vi "measure BT Hop Number.vi"(8 "error in (no error)":errorcluster, 11 "SA Measurement in":refnum<class "SA Measurement.lvclass">) -> (0 "error out":errorcluster, 3 "SA Measurement out":refnum<class "SA Measurement.lvclass">)   [LabVIEW 2023, in "Spectrum Analyzer.lvlib" / "SA Measurement.lvclass"]
uses:
  SA Measurement.lvclass
  SA Measurement.lvclass/SA Measurement.ctl
  TYPE DEFINITION/Keysight 9020A/TYPE Measurement Preset.ctl
  Spectrum Analyzer.lvlib
  TYPE DEFINITION/TYPE RBW and VBW Select.ctl
  Interface_Spectrum/Interface_Spectrum.lvclass
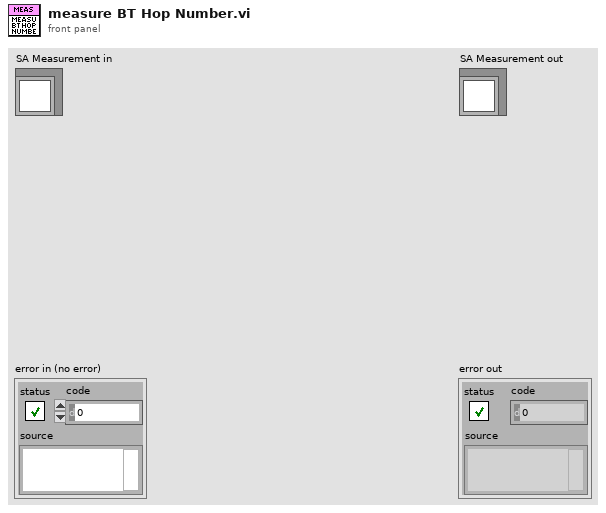
[diagram p1: front panel]
types:
  T1 = typedef "Spectrum Analyzer.lvlib/TYPE RBW and VBW Select.ctl" = enum16{"Res BW", "Video BW"}
  T2 = typedef "Spectrum Analyzer.lvlib/TYPE Measurement Preset.ctl" = enum16{"Sweep SA Mode", "Channel Power", "Occupied BW", "ACP", "Spurious Emission", "Spurious Emission Mask", "Burst Power (Transmit Power)"}
  T3 = typedef "Spectrum Analyzer.lvlib/TYPE Reference Level and Atten Param.ctl" = cluster{"Reference Level":dbl, "Atten":i32, "Atten Auto?":bool, "Reference Level Offset":dbl}
  T4 = typedef "Spectrum Analyzer.lvlib/TYPE Start and Stop Frequency.ctl" = cluster{"Start":dbl, "Stop":dbl}
  T5 = typedef "Spectrum Analyzer.lvlib/TYPE Display Trace Mode Select.ctl" = enum16{"Clear Write", "Max Hold", "Min Hold", "Average", "View"}
  T6 = typedef "Spectrum Analyzer.lvlib/TYPE Detect Mode Select.ctl" = enum16{"Det Auto (Normal)", "Auto Peak", "Positive Peak", "Negative Peak", "Sample", "RMS", "Average", "Quasipeak", "CISPR Average", "RMS Average"}
  T7 = cluster{"Trace Mode":T5, "Detector Type":T6, "Detect Auto?":bool}[]
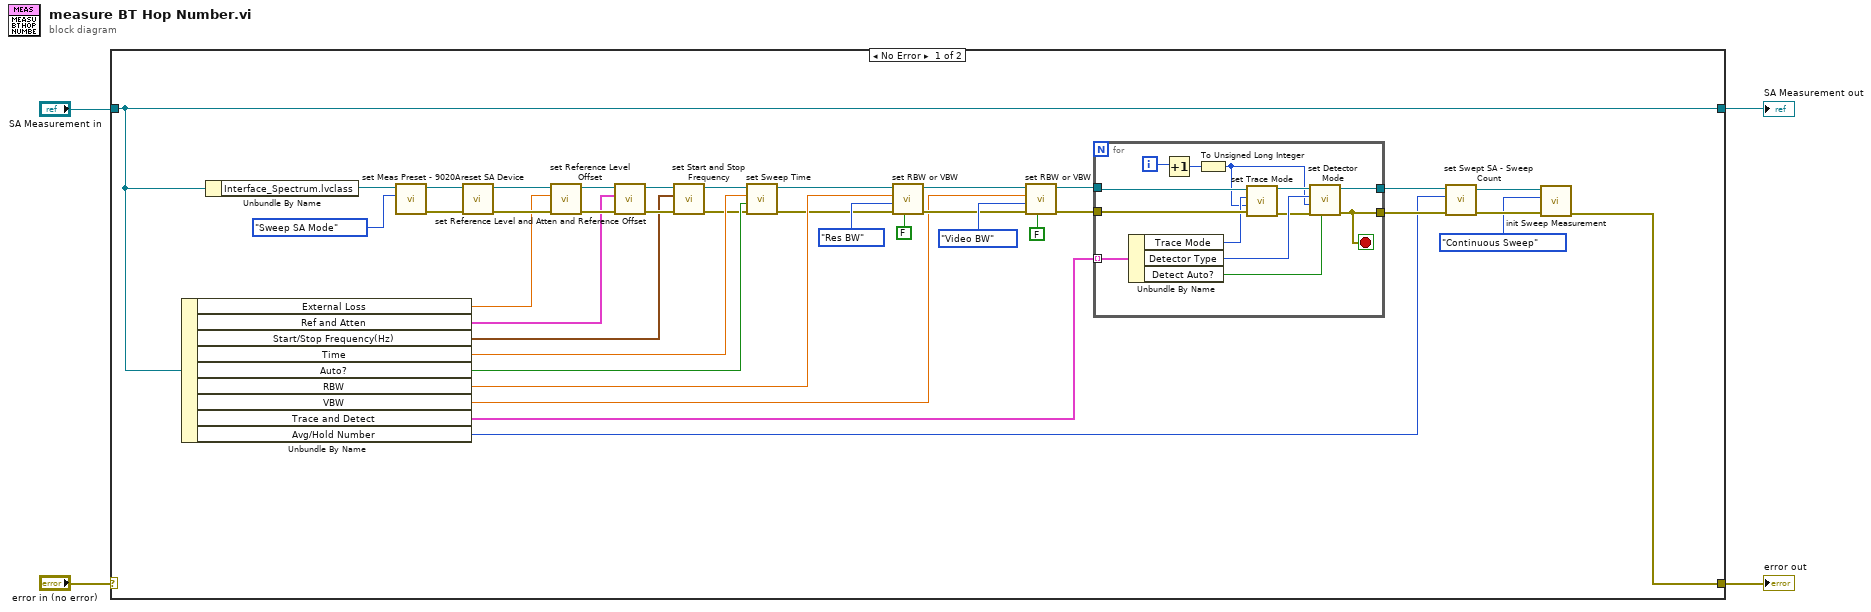
[diagram p0: block diagram]
diagram:
  n1 = case shown="No Error" "error in (no error)" {
    selector: "error in (no error)" -> [_ w57]
    tunnel: [w5 w57] -> w1
    tunnel: [w6 w56] -> w2
    tunnel: "SA Measurement in" -> [w6 w56]
    frame No Error {
      n2 = Unbundle By Name(w6) -> ("External Loss"=w34:dbl, "Ref and Atten"=w33:T3, "Start/Stop Frequency(Hz)"=w12:T4, "Time"=w18:dbl, "Auto?"=w17:bool, "RBW"=w26:dbl, "VBW"=w25:dbl, "Trace and Detect"=w22:T7, "Avg/Hold Number"=w19:u32)
      n3 = Unbundle By Name(w6) -> ("Interface_Spectrum.lvclass"=w42:refnum<class "Interface_Spectrum.lvclass">)
      n4 = call-dynamic "set Meas Preset - 9020A.vi"("Measurement Preset"=TYPE_Measurement_Preset."Sweep SA Mode", "Interface_Spectrum in"=w42) -> ("error out"=w39:errorcluster, "Interface_Spectrum out"=w40:refnum<class "Interface_Spectrum.lvclass">)  [unwired: 8 in]
      n5 = call-dynamic "reset SA Device.vi"("error in (no error)"=w39, "Interface_Spectrum in"=w40) -> ("error out"=w37:errorcluster, "Interface_Spectrum out"=w38:refnum<class "Interface_Spectrum.lvclass">)  [unwired: 8 in]
      n6 = call-dynamic "set Reference Level Offset.vi"("error in (no error)"=w37, "Reference Level Offset"=w34, "Interface_Spectrum in"=w38) -> ("error out"=w35:errorcluster, "Interface_Spectrum out"=w36:refnum<class "Interface_Spectrum.lvclass">)  [unwired: 7 in]
      n7 = call-dynamic "set Reference Level and Atten and Reference Offset.vi"("error in (no error)"=w35, "Reference Level, Atten, Reference Offset"=w33, "Interface_Spectrum in"=w36) -> ("error out"=w13:errorcluster, "Interface_Spectrum out"=w14:refnum<class "Interface_Spectrum.lvclass">)  [unwired: 7 in]
      n8 = call-dynamic "set Start and Stop Frequency.vi"("error in (no error)"=w13, "Start/Stop Frequency(Hz)"=w12, "Interface_Spectrum in"=w14) -> ("error out"=w10:errorcluster, "Interface_Spectrum out"=w11:refnum<class "Interface_Spectrum.lvclass">)  [unwired: 7 in]
      n9 = call-dynamic "set Sweep Time.vi"("error in (no error)"=w10, "Sweep Time Auto?"=w17, "Sweep Time(sec)"=w18, "Interface_Spectrum in"=w11) -> ("error out"=w15:errorcluster, "Interface_Spectrum out"=w16:refnum<class "Interface_Spectrum.lvclass">)  [unwired: 6 in]
      n10 = call-dynamic "set RBW or VBW.vi"("BW Auto?"=FALSE, "error in (no error)"=w15, "BW Type"=TYPE_RBW_and_VBW_Select."Res BW", "BW Value (Hz)"=w26, "Interface_Spectrum in"=w16) -> ("error out"=w27:errorcluster, "Interface_Spectrum out"=w28:refnum<class "Interface_Spectrum.lvclass">)  [unwired: 5 in]
      n11 = call-dynamic "set RBW or VBW.vi"("BW Auto?"=FALSE, "error in (no error)"=w27, "BW Type"=TYPE_RBW_and_VBW_Select."Video BW", "BW Value (Hz)"=w25, "Interface_Spectrum in"=w28) -> ("error out"=w23:errorcluster, "Interface_Spectrum out"=w24:refnum<class "Interface_Spectrum.lvclass">)  [unwired: 5 in]
      n12 = for {
        tunnel: w24 -> [w54]
        tunnel: w23 -> [w53]
        tunnel: w22 -> [w55] mode=indexing
        tunnel: [w43] -> w20
        tunnel: [w44] -> w21
        i -> [w52]
        stop <- w43 stop-if-true
        n13 = Unbundle By Name(w55) -> ("Trace Mode"=w50:T5, "Detector Type"=w48:T6, "Detect Auto?"=w45:bool)
        n14 = Increment(x=w52) -> (x+1=w51:i32)
        n15 = To Unsigned Long Integer(number=w51) -> (unsigned 32bit integer=w46:u32)
        n16 = call-dynamic "set Trace Mode.vi"("error in (no error)"=w53, "Trace Index"=w46, "Trace Mode"=w50, "Interface_Spectrum in"=w54) -> ("error out"=w47:errorcluster, "Interface_Spectrum out"=w49:refnum<class "Interface_Spectrum.lvclass">)  [unwired: 6 in]
        n17 = call-dynamic "set Detector Mode.vi"("Detect Auto?"=w45, "error in (no error)"=w47, "Trace Index"=w46, "Detector Type"=w48, "Interface_Spectrum in"=w49) -> ("error out"=w43:errorcluster, "Interface_Spectrum out"=w44:refnum<class "Interface_Spectrum.lvclass">)  [unwired: 5 in]
      }
      n18 = call-dynamic "set Swept SA - Sweep Count.vi"("error in (no error)"=w20, "Sweep Count"=w19, "Interface_Spectrum in"=w21) -> ("error out"=w8:errorcluster, "Interface_Spectrum out"=w9:refnum<class "Interface_Spectrum.lvclass">)  [unwired: 7 in]
      n19 = call-dynamic "init Sweep Measurement.vi"("error in (no error)"=w8, "Sweep Measurement Mode"=enum16{"Single Sweep", "Continuous Sweep"}."Continuous Sweep", "Interface_Spectrum in"=w9) -> ("error out"=w5:errorcluster)  [unwired: 7 in, 1 out]
    }
    frame Error {
    }
  }
  "error out" <- w1
  "SA Measurement out" <- w2
